vi "ControllerUI_New.vi"() -> ()   [LabVIEW 2026]
uses:
  <userlib>/_OpenG.lib/file/file.llb/openg_file.lvlib
panel:
  in  "BTN_Wind_Turbine":bool
  out "background":picture
  in  "Tab Control":T1(tab)
  in  "Mode 4":bool
  in  "Mode 3":bool
  in  "Mode 2":bool
  in  "Mode 1":bool
  in  "WT Wind Speed":dbl min=0.0 max=30.0 step=0.5
  in  "stop":bool
  out "Local Status":string
  in  "WT PWM Command":dbl min=0.0 max=255.0 step=1.0
  out "Last Update":string
  out "UDP Frame":string
  out "Active Power":string
  out "Current":string
  out "Voltage":string
  in  "Reset Node":bool
  in  "Read Device State":bool
  in  "Send UDP Command":bool
  in  "LED Flow Speed":dbl min=0.0 max=80.0 step=1.0
  in  "Voltage Command":dbl min=0.0 max=255.0 step=1.0
  in  "Node Enable":bool
  out "Device Badge":string
  out "Selected Summary":string
  out "Device Description":string
  out "Node ID":string
  out "Device Name":string
  # "Preset Disaster Mode"
  # "Selected Node Telemetry"
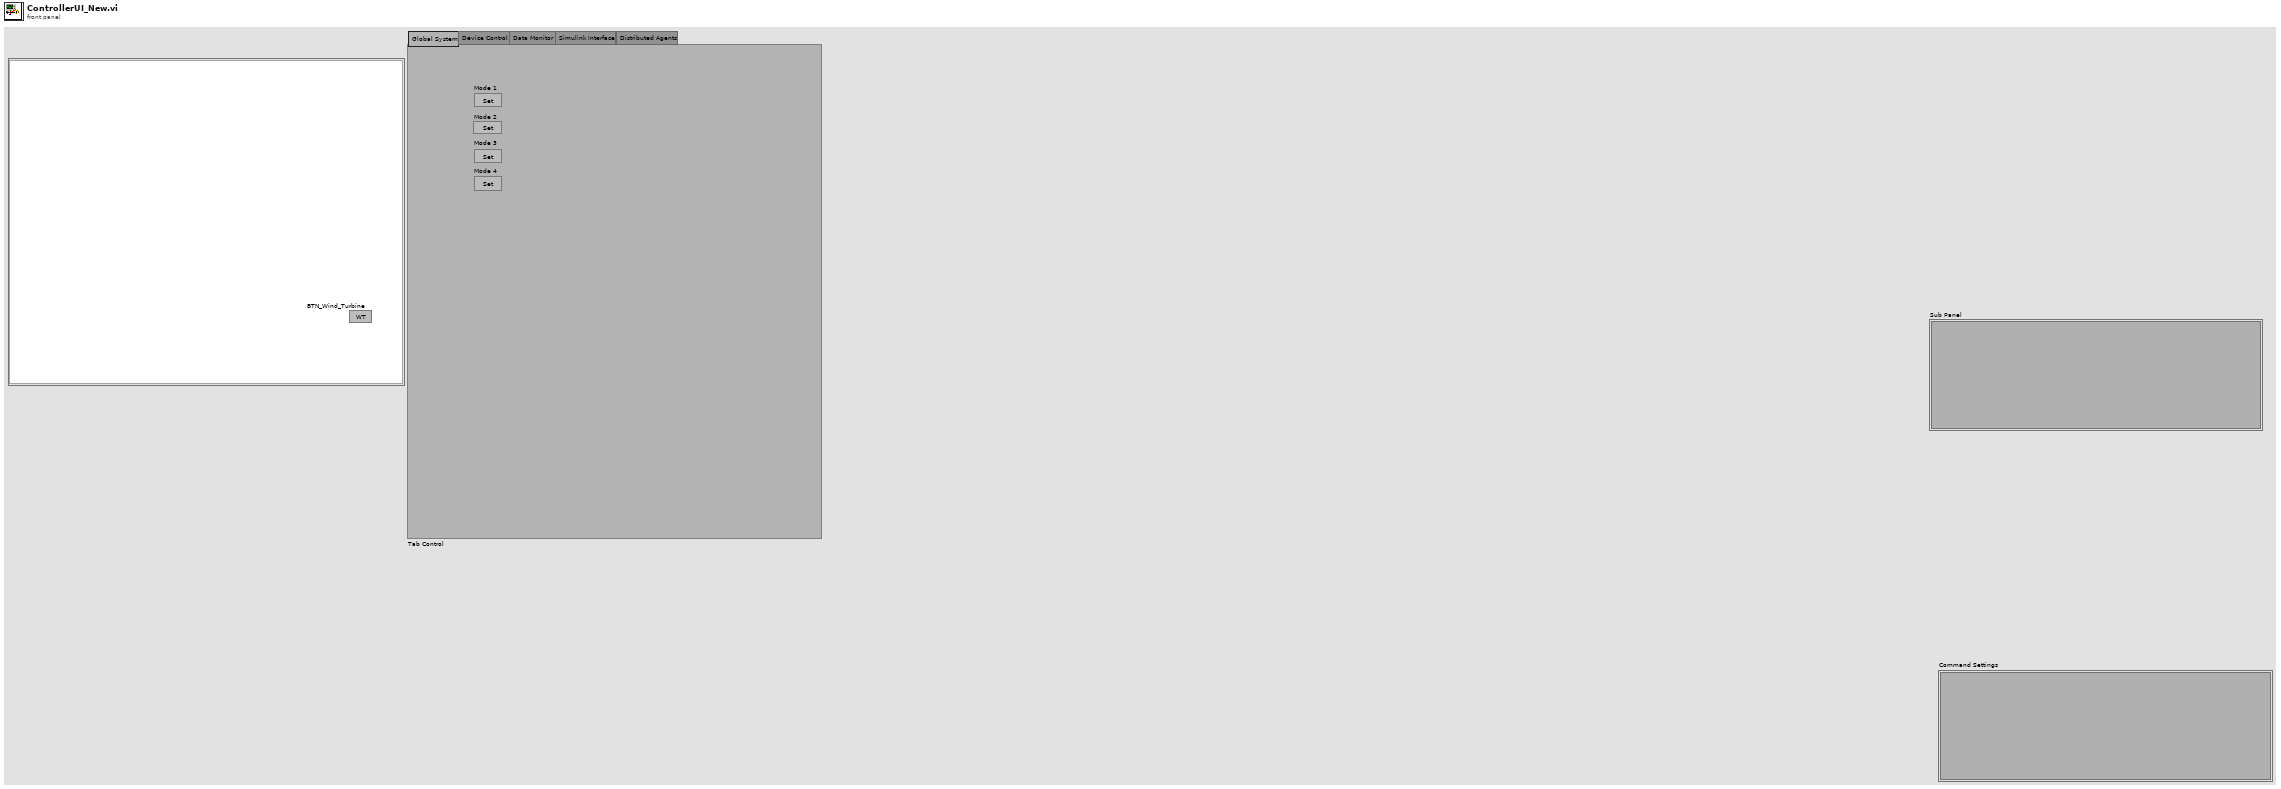
[diagram p1: front panel]
types:
  T1 = enum32{"Global System", "Device Control", "Data Monitor", "Simulink Interface", "Distributed Agents"}
  T2 = typedef "imagedata.ctl" = cluster{"image type":i32, "image depth":i32, "image":u8[], "mask":u8[], "colors":u32[], "Rectangle":cluster{"left":i16, "top":i16, "right":i16, "bottom":i16}}
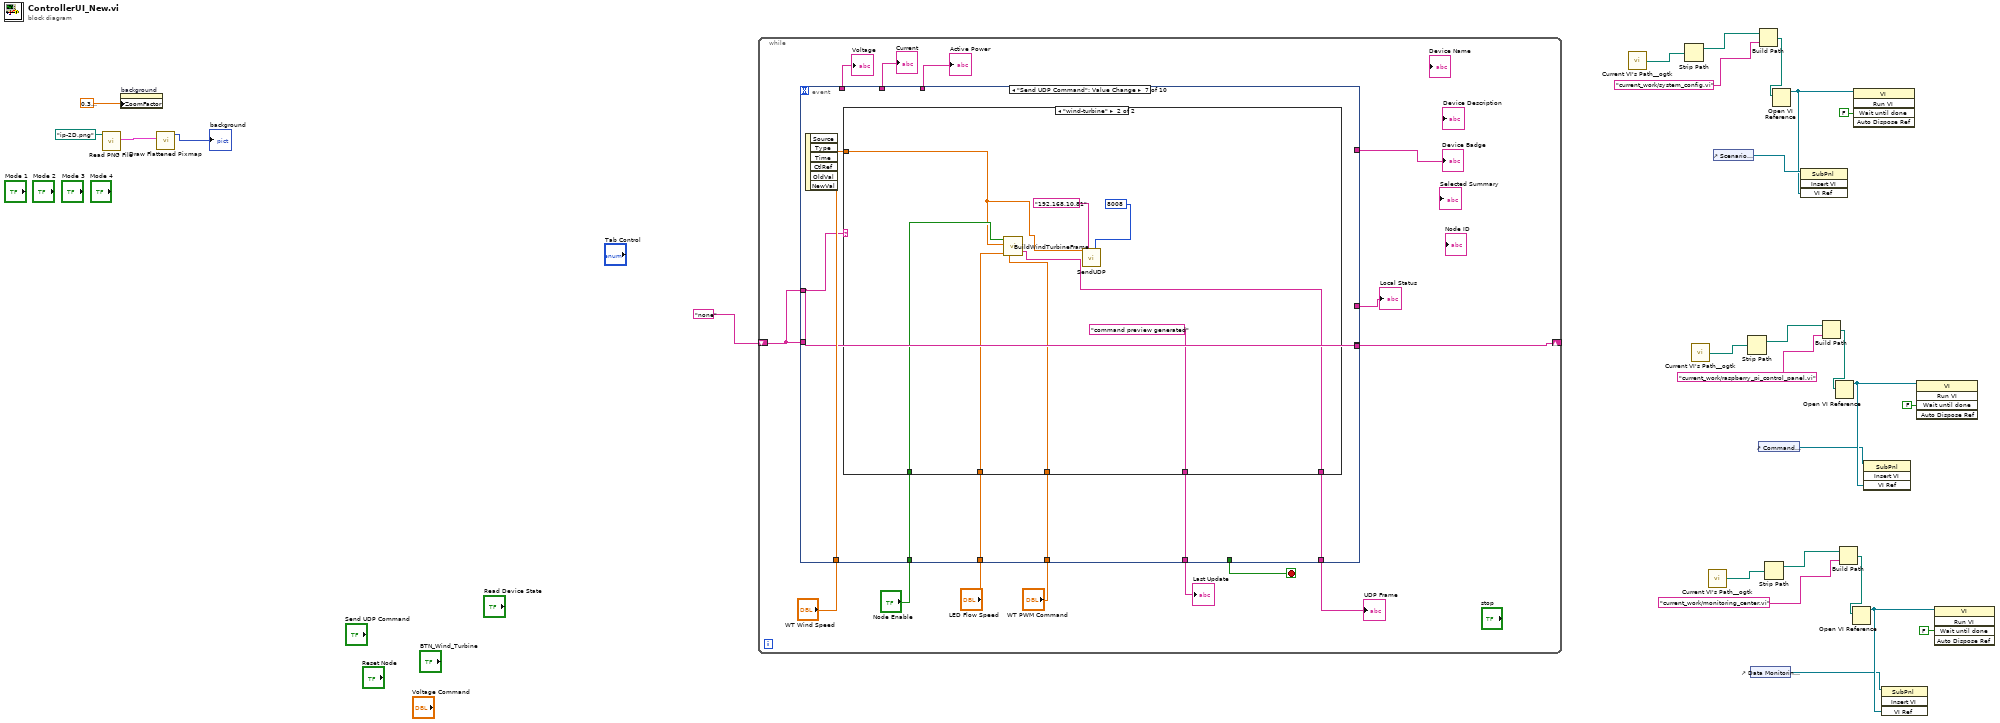
[diagram p0: block diagram]
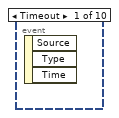
[diagram p2: hidden frame]
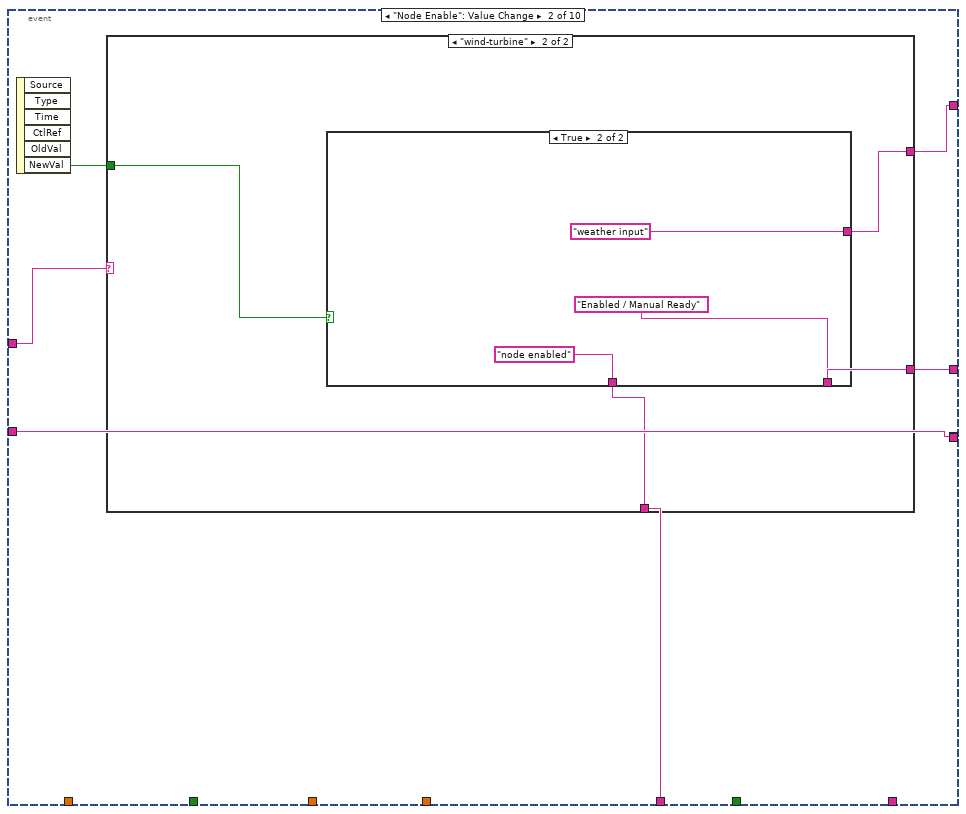
[diagram p3: hidden frame]
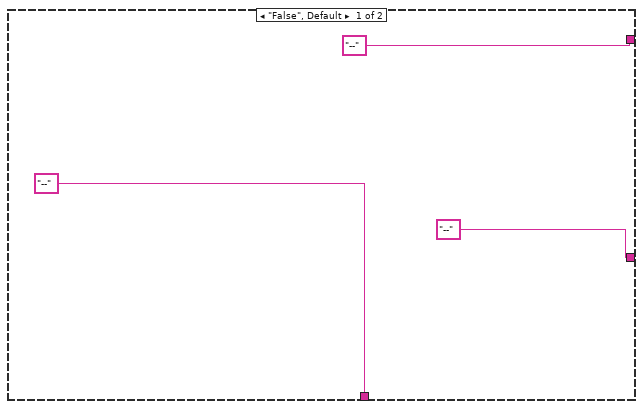
[diagram p4: hidden frame]
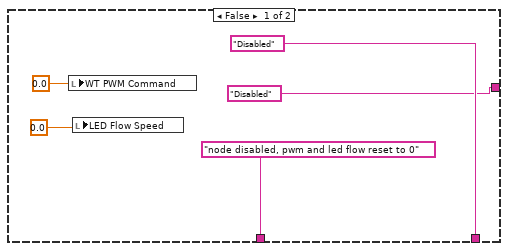
[diagram p5: hidden frame]
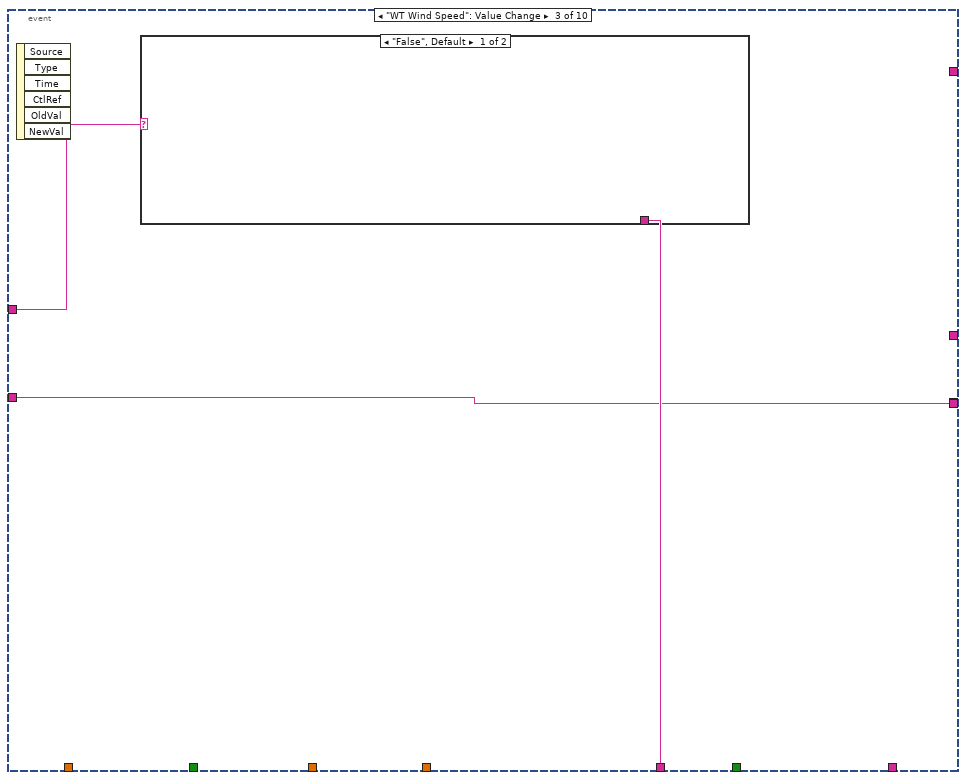
[diagram p6: hidden frame]
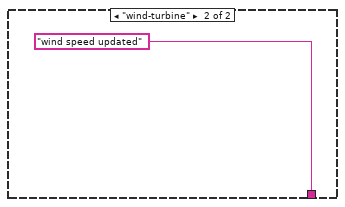
[diagram p7: hidden frame]
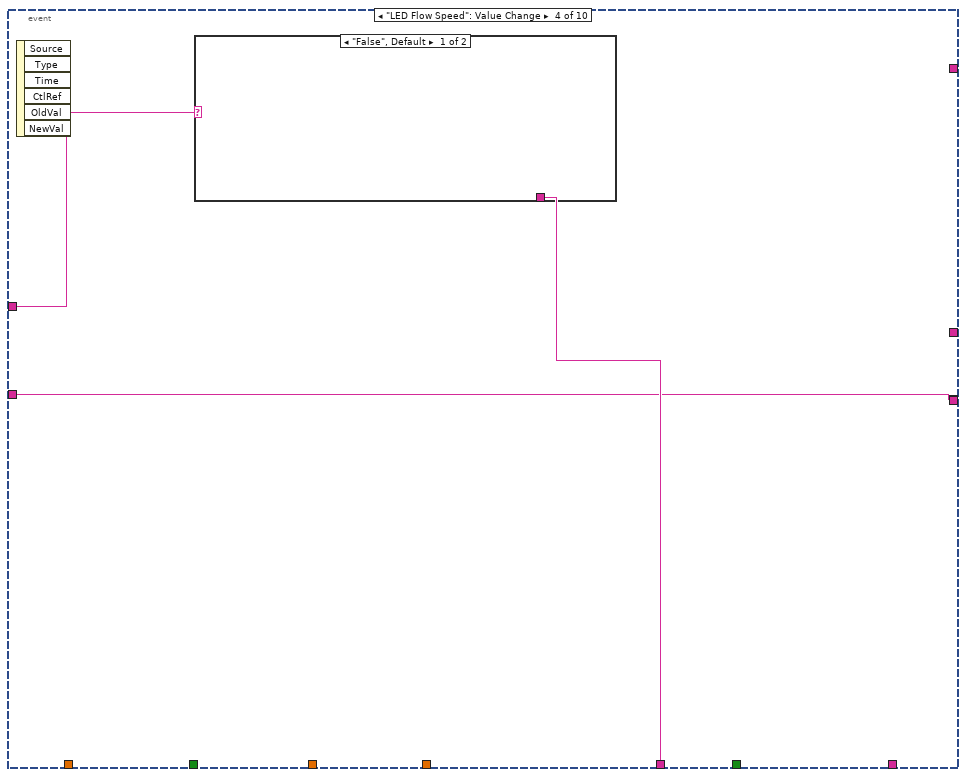
[diagram p8: hidden frame]
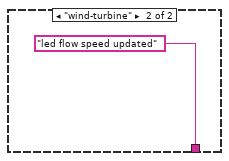
[diagram p9: hidden frame]
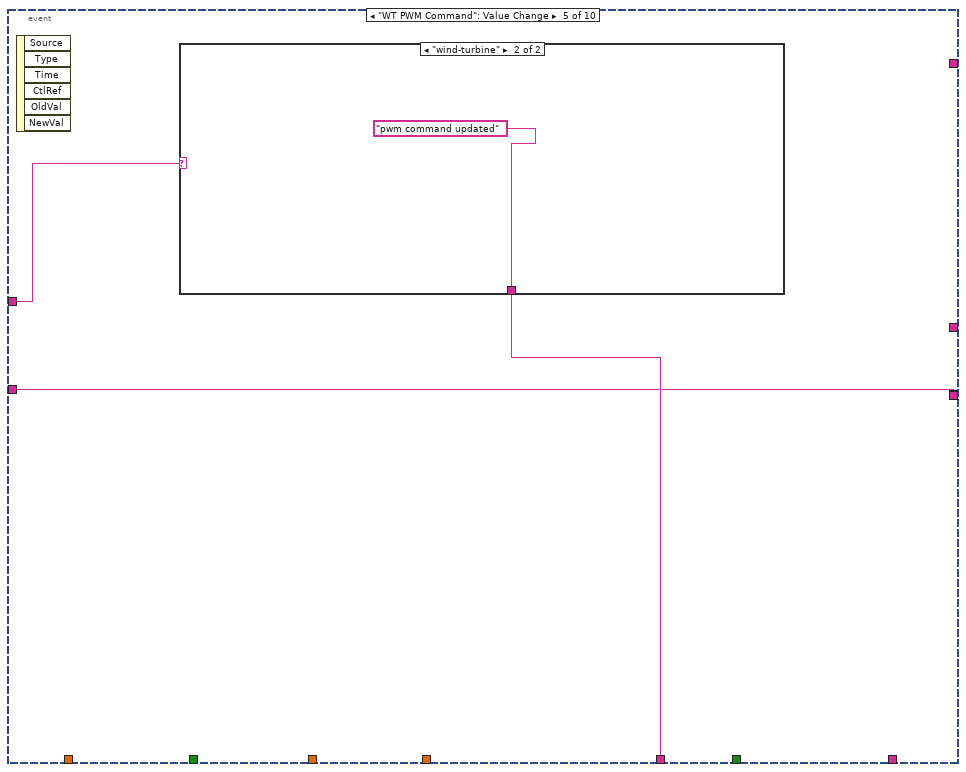
[diagram p10: hidden frame]
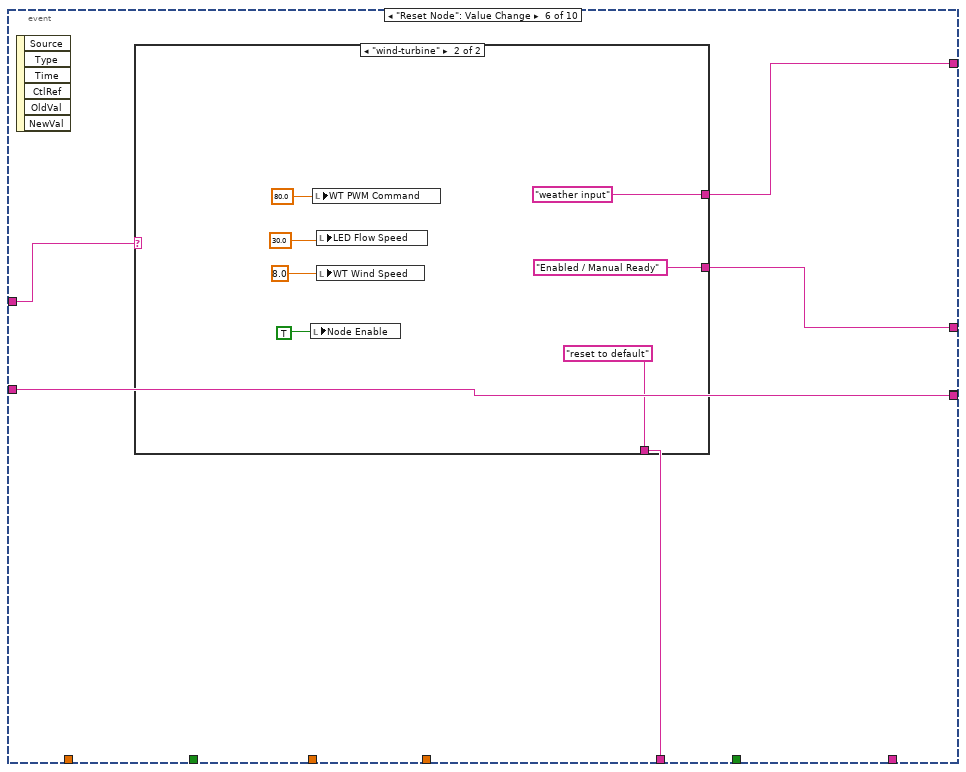
[diagram p12: hidden frame]
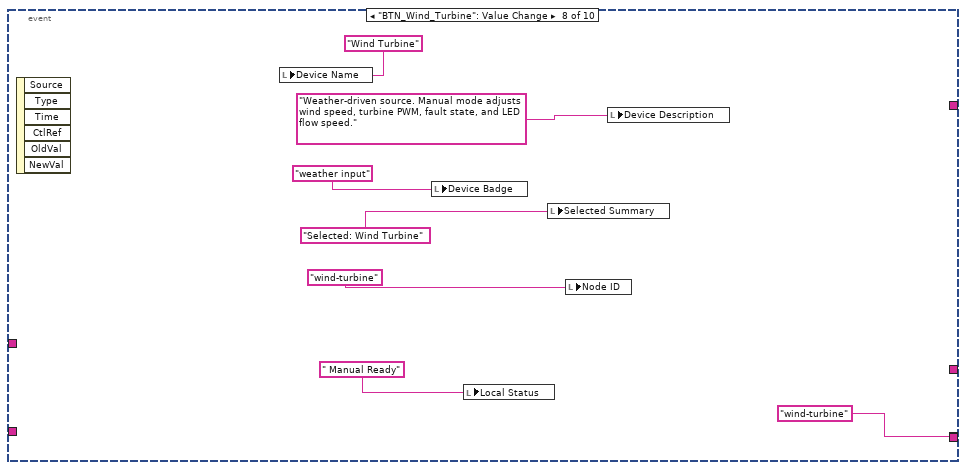
[diagram p15: hidden frame]
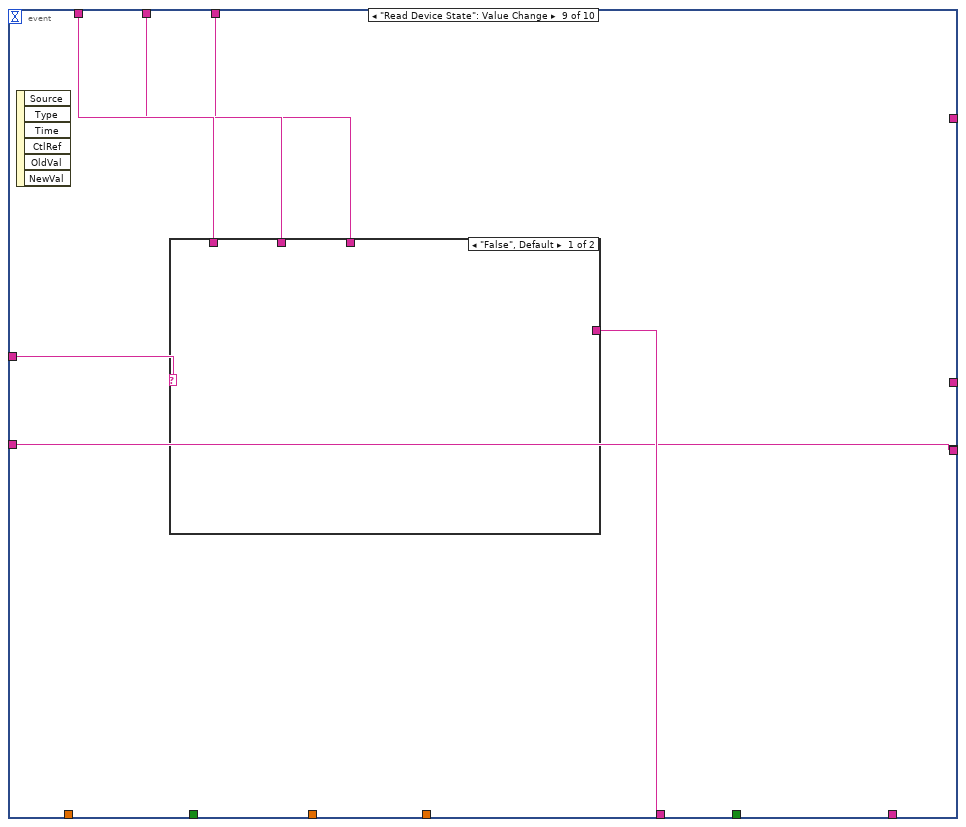
[diagram p16: hidden frame]
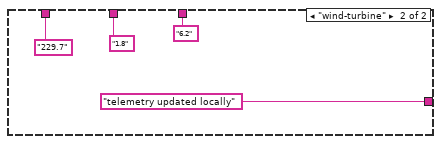
[diagram p17: hidden frame]
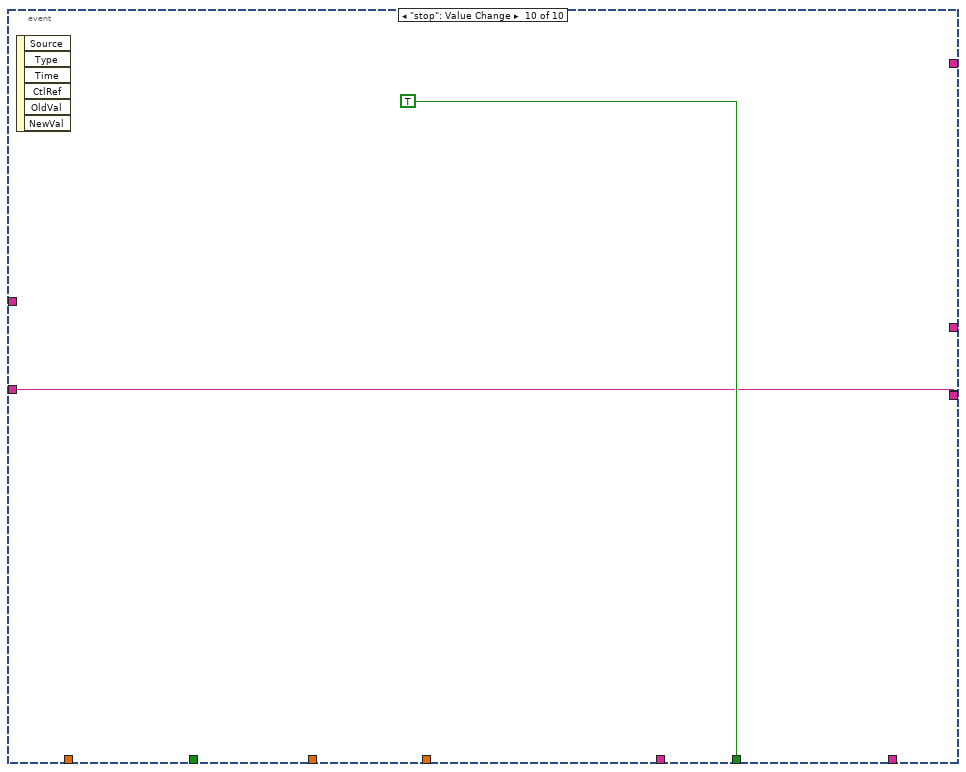
[diagram p18: hidden frame]
diagram:
  n1 = call <vilib>:"Read PNG File.vi"("path to PNG file"=path "ip-2D.png") -> ("image data"=w26:T2)  [unwired: 8 in, 2 out]
  n2 = property on="background" class="Pict"("ZoomFactor"=sgl 0.3 ("Zoom Factor")) -> ()  [unwired: 2 in, 2 out]
  n3 = call <vilib>:"Draw Flattened Pixmap.vi"("image data"=w26) -> ("new picture"=→"background":picture)  [unwired: 8 in]
  n4 = while {
    shift-right: [w28] -> _
    shift-left: "none" -> [w27]
    stop <- w40 stop-if-true
    n5 = event shown="[6] \"Send UDP Command\": Value Change" {
      selector: _ -> [_ _ _ _ _ _ _ _ _ _]
      dyn-events: _ -> [_ _ _ _ _ _ _ _ _ _]
      timeout: _ -> [_ _ _ _ _ _ _ _ _ _]
      tunnel: [_ _ _ _ _ _ _ _ _ TRUE] -> w40
      tunnel: [_ w44 _ _ _ w77 _ _ _ _] -> w38
      tunnel: [_ w43 _ _ _ w76 _ _ _ _] -> w39
      tunnel: [_ w45 w64 w68 w72 w78 w87 _ w113 _] -> w37
      tunnel: "Node Enable" -> [_ _ _ _ _ _ w92 _ _ _]
      tunnel: "WT Wind Speed" -> [_ _ _ _ _ _ w91 _ _ _]
      tunnel: "WT PWM Command" -> [_ _ _ _ _ _ w90 _ _ _]
      tunnel: "LED Flow Speed" -> [_ _ _ _ _ _ w89 _ _ _]
      tunnel: [_ _ _ _ _ _ w88 _ _ _] -> w32
      tunnel: [_ _ _ _ _ _ _ _ w112 _] -> w31
      tunnel: [_ _ _ _ _ _ _ _ w111 _] -> w30
      tunnel: [_ _ _ _ _ _ _ _ w110 _] -> w29
      tunnel: [_ w41 _ w66 w70 _ w86 "wind-turbine" w108 w118] -> w28
      tunnel: w27 -> [_ w42 w63 w67 w71 w75 w86 _ w109 _]
      tunnel: w27 -> [_ w41 w62 w66 w70 w74 _ _ w108 w118]
      tunnel: [_ _ w62 _ _ _ _ _ _ _] -> _
      tunnel: [_ _ _ _ _ w74 _ _ _ _] -> _
      event Timeout {
        n6 = event-data() -> ()  [unwired: 1 in, 3 out]
      }
      event "Node Enable": Value Change {
        n7 = event-data() -> ("NewVal"=w46:bool)  [unwired: 1 in, 5 out]
        n8 = case shown="\"wind-turbine\"" w42 {
          tunnel: w46 -> [_ w53]
          tunnel: ["--" w52] -> w45
          tunnel: ["--" w51] -> w44
          tunnel: ["--" w50] -> w43
          frame "False", Default {
          }
          frame "wind-turbine" {
            n9 = case shown="True" w53 {
              tunnel: ["node disabled, pwm and led flow reset to 0" "node enabled"] -> w52
              tunnel: ["Disabled" "Enabled / Manual Ready"] -> w51
              tunnel: ["Disabled" "weather input"] -> w50
              frame False {
                n10 = local write "WT PWM Command"(0.0 ("WT PWM Command")) -> ()
                n11 = local write "LED Flow Speed"(0.0 ("WT Wind Speed")) -> ()
              }
              frame True {
              }
            }
          }
        }
      }
      event "WT Wind Speed": Value Change {
        n12 = event-data() -> ()  [unwired: 1 in, 6 out]
        n13 = case shown="\"False\", Default" w63 {
          tunnel: [_ "wind speed updated"] -> w64
          frame "False", Default {
          }
          frame "wind-turbine" {
          }
        }
      }
      event "LED Flow Speed": Value Change {
        n14 = event-data() -> ()  [unwired: 1 in, 6 out]
        n15 = case shown="\"False\", Default" w67 {
          tunnel: [_ "led flow speed updated"] -> w68
          frame "False", Default {
          }
          frame "wind-turbine" {
          }
        }
      }
      event "WT PWM Command": Value Change {
        n16 = event-data() -> ()  [unwired: 1 in, 6 out]
        n17 = case shown="\"wind-turbine\"" w71 {
          tunnel: [_ "pwm command updated"] -> w72
          frame "False", Default {
          }
          frame "wind-turbine" {
          }
        }
      }
      event "Reset Node": Value Change {
        n18 = event-data() -> ()  [unwired: 1 in, 6 out]
        n19 = case shown="\"wind-turbine\"" w75 {
          tunnel: [_ "reset to default"] -> w78
          tunnel: [_ "Enabled / Manual Ready"] -> w77
          tunnel: [_ "weather input"] -> w76
          frame "False", Default {
          }
          frame "wind-turbine" {
            n20 = local write "Node Enable"(TRUE ("Node Enable")) -> ()
            n21 = local write "WT PWM Command"(80.0 ("WT PWM Command")) -> ()
            n22 = local write "LED Flow Speed"(30.0 ("WT Wind Speed")) -> ()
            n23 = local write "WT Wind Speed"(8.0 ("WT PWM Command")) -> ()
          }
        }
      }
      event "Send UDP Command": Value Change {
        n24 = event-data() -> ()  [unwired: 1 in, 6 out]
        n25 = case shown="\"wind-turbine\"" w86 {
          tunnel: w92 -> [_ w99]
          tunnel: w91 -> [_ w94]
          tunnel: w90 -> [_ w95]
          tunnel: w89 -> [_ w98]
          tunnel: [_ w93] -> w88
          tunnel: [_ "command preview generated"] -> w87
          frame "False", Default {
          }
          frame "wind-turbine" {
            n26 = call "BuildWindTurbineFrame.vi"("LED Flow Speed"=w98, "PWM Command"=w95, "Wind Speed"=w94, "Node Enable"=w99) -> ("Frame Preview"=w93:string)  [unwired: 1 out]
            n27 = call "SendUDP.vi"("Arg3"=w94, "IP"="192.168.10.81", "Port"=8008) -> ()  [unwired: 13 in]
          }
        }
      }
      event "BTN_Wind_Turbine": Value Change {
        n28 = event-data() -> ()  [unwired: 1 in, 6 out]
        n29 = local write "Device Name"("Wind Turbine") -> ()
        n30 = local write "Device Badge"("weather input") -> ()
        n31 = local write "Local Status"(" Manual Ready") -> ()
        n32 = local write "Selected Summary"("Selected: Wind Turbine") -> ()
        n33 = local write "Node ID"("wind-turbine") -> ()
        n34 = local write "Device Description"("Weather-driven source. Manual mode adjusts wind speed, turbine PWM, fault state, and LED flow speed.") -> ()
      }
      event "Read Device State": Value Change {
        n35 = event-data() -> ()  [unwired: 1 in, 6 out]
        n36 = case shown="\"False\", Default" w109 {
          tunnel: [_ "telemetry updated locally"] -> w113
          tunnel: [_ "229.7"] -> w112
          tunnel: [_ "1.8"] -> w111
          tunnel: [_ "6.2"] -> w110
          frame "False", Default {
          }
          frame "wind-turbine" {
          }
        }
      }
      event "stop": Value Change {
        n37 = event-data() -> ()  [unwired: 1 in, 6 out]
      }
    }
    "Local Status" <- w38
    "Device Badge" <- w39
    "Last Update" <- w37
    "UDP Frame" <- w32
    "Voltage" <- w31
    "Current" <- w30
    "Active Power" <- w29
  }
  n38 = call <userlib>:"Current VI's Path__ogtk.vi"() -> ("Current VI's Path (+ Relative)"=w18:path)  [unwired: 1 in]
  n39 = Strip Path(path=w18) -> (stripped path=w17:path)  [unwired: 1 out]
  n40 = call <userlib>:"Current VI's Path__ogtk.vi"() -> ("Current VI's Path (+ Relative)"=w12:path)  [unwired: 1 in]
  n41 = call <userlib>:"Current VI's Path__ogtk.vi"() -> ("Current VI's Path (+ Relative)"=w5:path)  [unwired: 1 in]
  n42 = control-ref of="Scenario Parameters Settings"() -> (w21:refnum<vi>)
  n43 = Strip Path(path=w12) -> (stripped path=w11:path)  [unwired: 1 out]
  n44 = control-ref of="Data Monitoring Center"() -> (w1:refnum<vi>)
  n45 = control-ref of="Command Settings"() -> (w8:refnum<vi>)
  n46 = Build Path(base path=w17, name or relative path="current_work/system_config.vi") -> (appended path=w15:path)
  n47 = Strip Path(path=w5) -> (stripped path=w4:path)  [unwired: 1 out]
  n48 = Open VI Reference(vi path=w15) -> (vi reference=w20:refnum<vi>)  [unwired: 5 in, 1 out]
  n49 = invoke class="SubPnl" method="Insert VI"(reference=w21, "VI Ref"=w20) -> ()  [unwired: 2 in, 4 out]
  n50 = Build Path(base path=w11, name or relative path="current_work/raspberry_pi_control_panel.vi") -> (appended path=w9:path)
  n51 = Open VI Reference(vi path=w9) -> (vi reference=w14:refnum<vi>)  [unwired: 5 in, 1 out]
  n52 = Build Path(base path=w4, name or relative path="current_work/monitoring_center.vi") -> (appended path=w2:path)
  n53 = Open VI Reference(vi path=w2) -> (vi reference=w7:refnum<vi>)  [unwired: 5 in, 1 out]
  n54 = invoke class="VI" method="Run VI"(reference=w20, "Wait until done"=FALSE ("Wait Until Done")) -> ()  [unwired: 3 in, 5 out]
  n55 = invoke class="SubPnl" method="Insert VI"(reference=w8, "VI Ref"=w14) -> ()  [unwired: 2 in, 4 out]
  n56 = invoke class="SubPnl" method="Insert VI"(reference=w1, "VI Ref"=w7) -> ()  [unwired: 2 in, 4 out]
  n57 = invoke class="VI" method="Run VI"(reference=w14, "Wait until done"=FALSE ("Wait Until Done")) -> ()  [unwired: 3 in, 5 out]
  n58 = invoke class="VI" method="Run VI"(reference=w7, "Wait until done"=FALSE ("Wait Until Done")) -> ()  [unwired: 3 in, 5 out]
